vi "test Import Configuration File.vi"(8 "error in":errorcluster, 11 "TestCase in":refnum<class "Import.lvclass">) -> (0 "error out":errorcluster, 3 "TestCase out":refnum<class "Import.lvclass">)   [LabVIEW 2020, in "Import.lvclass"]
uses:
  Import.lvclass
  Import.lvclass/Import.ctl
  C:/Program Files/National Instruments/LabVIEW 2026/vi.lib/addons/_JKI Toolkits/VI Tester/TestCase.llb/TestCase.lvclass
  <vilib>/addons/_JKI Toolkits/VI Tester/TestCase.llb/TestCase.lvclass
  Import/ARINC 429 Import.lvlib
  <userlib>/_OpenG.lib/appcontrol/appcontrol.llb/openg_application_control.lvlib
  <vilib>/NI/VeriStand Custom Device Testing Tools/VeriStandTestUtilities/VeriStandTestUtilities.lvlib
  Shared/Transfer Type.ctl
  Shared/Direction.ctl
  Shared/Transfer Speed.ctl
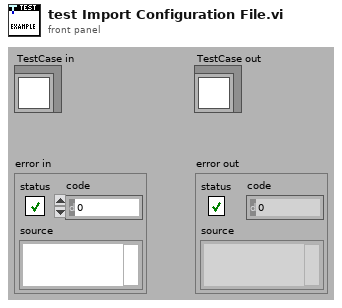
[diagram p1: front panel]
types:
  T1 = typedef "Direction.ctl" = enum16{"Rx", "Tx"}
  T2 = typedef "Transfer Type.ctl" = enum16{"Scheduled", "Acyclic", "Block", "Strobe"}
  T3 = typedef "Transfer Speed.ctl" = enum16{"LO (12.5 kb/s)", "HI (100 kb/s)"}
  T4 = cluster{"hardware channel":i32, "direction":T1, "labels":cluster{"label (Dec)":i32, "parameters":cluster{"name":string, "unit":string, "Parameter":cluster{"start index":i32, "size":i32, "encoding":enum16{"BNR", "BCD", "Discrete"}, "signed":bool, "scale multiplier":dbl, "scale offset":dbl, "default value":dbl}}[], "SDI value":u8, "SDI enabled":bool, "transfer type":T2, "SDI enabled 2":bool, "transmit period":u32}[], "speed":T3}[]
  T5 = typedef "VS Channels Definition for All Labels on Hardware Channel.ctl" = cluster{"hardware channel":i32, "direction":T1, "labels":T6[], "speed":T3}
  T6 = typedef "VS Channels Definition for Label.ctl" = cluster{"label (Dec)":u32, "parameters":T7[], "SDI value":u8, "SDI enabled":bool, "transfer type":T2, "create timestamp":bool, "transmit period":u32}
  T7 = typedef "VS Channel Definition for Parameter.ctl" = cluster{"name":string, "unit":string, "Parameter":T8}
  T8 = typedef "Parameter Definition.ctl" = cluster{"start index":i32, "size":i32, "encoding":T9, "signed":bool, "scale multiplier":dbl, "scale offset":dbl, "default value":dbl}
  T9 = typedef "Encoding and Decoding.lvlib/Encoding.ctl" = enum16{"BNR", "BCD", "Discrete"}
  T10 = cluster{"hardware channel":i32, "direction":T1, "labels":cluster{"label (Dec)":i32, "parameters":cluster{"name":string, "unit":string, "Parameter":cluster{"start index":i32, "size":i32, "encoding":enum16{"BNR", "BCD", "Discrete"}, "signed":bool, "scale multiplier":dbl, "scale offset":dbl, "default value":dbl}}[], "SDI value":u8, "SDI enabled":bool, "transfer type":T2, "SDI enabled 2":bool, "transmit period":u32}[], "speed":T3}
  T11 = cluster{"label (Dec)":i32, "parameters":cluster{"name":string, "unit":string, "Parameter":cluster{"start index":i32, "size":i32, "encoding":enum16{"BNR", "BCD", "Discrete"}, "signed":bool, "scale multiplier":dbl, "scale offset":dbl, "default value":dbl}}[], "SDI value":u8, "SDI enabled":bool, "transfer type":T2, "SDI enabled 2":bool, "transmit period":u32}[]
  T12 = cluster{"label (Dec)":i32, "parameters":cluster{"name":string, "unit":string, "Parameter":cluster{"start index":i32, "size":i32, "encoding":enum16{"BNR", "BCD", "Discrete"}, "signed":bool, "scale multiplier":dbl, "scale offset":dbl, "default value":dbl}}[], "SDI value":u8, "SDI enabled":bool, "transfer type":T2, "SDI enabled 2":bool, "transmit period":u32}
  T13 = cluster{"name":string, "unit":string, "Parameter":cluster{"start index":i32, "size":i32, "encoding":enum16{"BNR", "BCD", "Discrete"}, "signed":bool, "scale multiplier":dbl, "scale offset":dbl, "default value":dbl}}[]
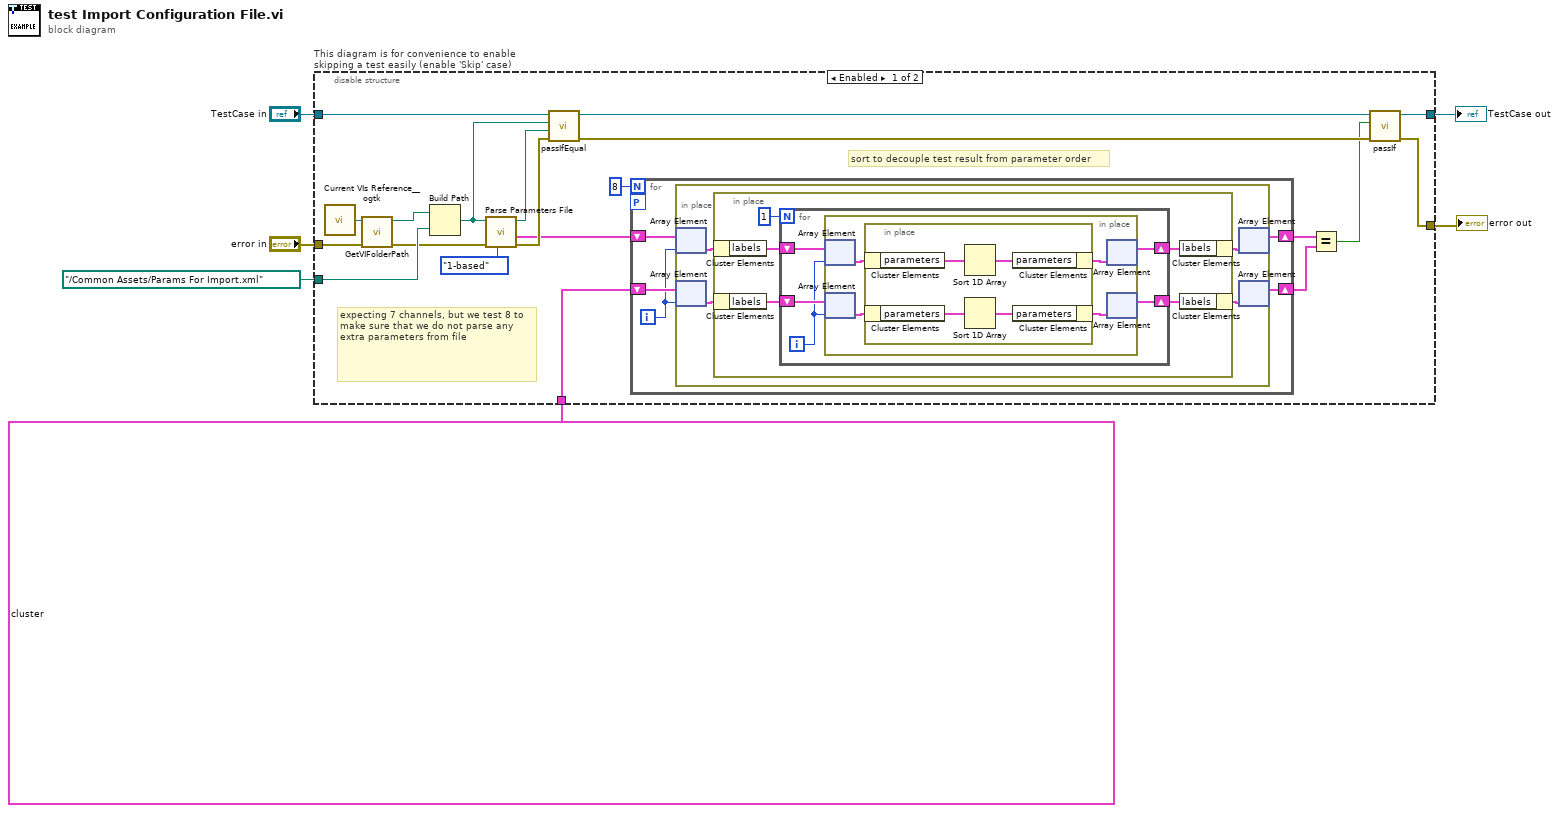
[diagram p0: block diagram]
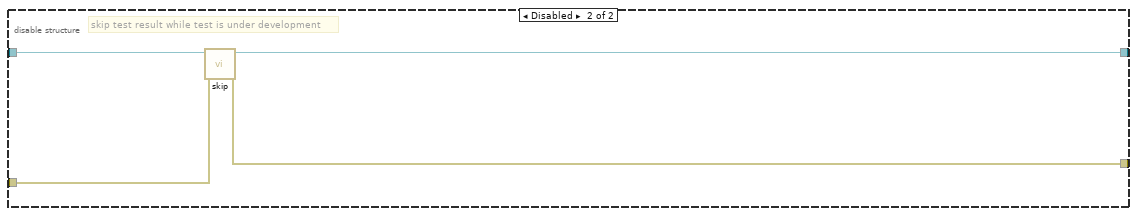
[diagram p2: hidden frame]
diagram:
  n1 = disable-structure "This diagram is for convenience to enable skipping a test easily (enable 'Skip' case)" shown="Enabled" {
    disable-tunnel: "TestCase in" -> [w26 w57]
    disable-tunnel: [w15 w55] -> w3
    disable-tunnel: [w16 w56] -> w5
    disable-tunnel: "error in" -> [w23 w54]
    disable-tunnel: path "../Common Assets/Params For Import.xml" ("Absolute or Relative Path") -> [w22 _]
    disable-tunnel: T4 [{"hardware channel"=1, "direction"=enum."Rx", "labels"=[{"label (Dec)"=134, "parameters"=[{"name"="Altitude_Rx", "unit"="psi", "Parameter"={"start index"=18, "size"=10, "encoding"=enum."BNR", "signed"=TRUE, "scale multiplier"=16.0, "scale offset"=0.0, "default value"=0.0}}, {"name"="SSM", "unit"="", "Parameter"={"start index"=29, "size"=2, "encoding"=enum."BNR", "signed"=FALSE, "scale multiplier"=1.0, "scale offset"=0.0, "default value"=0.0}}, {"name"="Parity", "unit"="", "Parameter"={"start index"=31, "size"=1, "encoding"=enum."Discrete", "signed"=FALSE, "scale multiplier"=1.0, "scale offset"=0.0, "default value"=0.0}}], "SDI value"=4, "SDI enabled"=FALSE, "transfer type"=enum."Scheduled", "SDI enabled 2"=TRUE, "transmit period"=1000}], "speed"=enum."LO (12.5 kb/s)"}, {"hardware channel"=2, "direction"=enum."Rx", "labels"=[{"label (Dec)"=135, "parameters"=[{"name"="Altitude_Rx", "unit"="ft", "Parameter"={"start index"=10, "size"=19, "encoding"=enum."BCD", "signed"=TRUE, "scale multiplier"=1.0, "scale offset"=0.0, "default value"=0.0}}, {"name"="SSM", "unit"="", "Parameter"={"start index"=29, "size"=2, "encoding"=enum."BNR", "signed"=FALSE, "scale multiplier"=1.0, "scale offset"=0.0, "default value"=0.0}}], "SDI value"=2, "SDI enabled"=TRUE, "transfer type"=enum."Scheduled", "SDI enabled 2"=FALSE, "transmit period"=1000}], "speed"=enum."HI (100 kb/s)"}, {"hardware channel"=4, "direction"=enum."Rx", "labels"=[{"label (Dec)"=136, "parameters"=[{"name"="Altitude_Rx", "unit"="m", "Parameter"={"start index"=13, "size"=16, "encoding"=enum."BNR", "signed"=TRUE, "scale multiplier"=1.0, "scale offset"=0.0, "default value"=0.0}}, {"name"="valid_Rx", "unit"="", "Parameter"={"start index"=10, "size"=1, "encoding"=enum."Discrete", "signed"=FALSE, "scale multiplier"=1.0, "scale offset"=0.0, "default value"=0.0}}, {"name"="current_Rx", "unit"="", "Parameter"={"start index"=11, "size"=1, "encoding"=enum."Discrete", "signed"=FALSE, "scale multiplier"=1.0, "scale offset"=0.0, "default value"=0.0}}, {"name"="SSM", "unit"="", "Parameter"={"start index"=29, "size"=2, "encoding"=enum."BNR", "signed"=FALSE, "scale multiplier"=1.0, "scale offset"=0.0, "default value"=0.0}}], "SDI value"=4, "SDI enabled"=FALSE, "transfer type"=enum."Scheduled", "SDI enabled 2"=FALSE, "transmit period"=1000}], "speed"=enum."HI (100 kb/s)"}, {"hardware channel"=17, "direction"=enum."Tx", "labels"=[{"label (Dec)"=134, "parameters"=[{"name"="Altitude_Tx", "unit"="psi", "Parameter"={"start index"=18, "size"=10, "encoding"=enum."BNR", "signed"=TRUE, "scale multiplier"=16.0, "scale offset"=0.0, "default value"=0.0}}], "SDI value"=4, "SDI enabled"=FALSE, "transfer type"=enum."Scheduled", "SDI enabled 2"=FALSE, "transmit period"=20000}], "speed"=enum."HI (100 kb/s)"}, {"hardware channel"=19, "direction"=enum."Tx", "labels"=[{"label (Dec)"=135, "parameters"=[{"name"="Altitude_Tx", "unit"="ft", "Parameter"={"start index"=10, "size"=19, "encoding"=enum."BCD", "signed"=TRUE, "scale multiplier"=1.0, "scale offset"=0.0, "default value"=0.0}}], "SDI value"=2, "SDI enabled"=TRUE, "transfer type"=enum."Scheduled", "SDI enabled 2"=FALSE, "transmit period"=50000}], "speed"=enum."HI (100 kb/s)"}, {"hardware channel"=21, "direction"=enum."Tx", "labels"=[{"label (Dec)"=136, "parameters"=[{"name"="Altitude_Tx", "unit"="m", "Parameter"={"start index"=13, "size"=16, "encoding"=enum."BNR", "signed"=TRUE, "scale multiplier"=1.0, "scale offset"=0.0, "default value"=0.0}}, {"name"="valid_Tx", "unit"="", "Parameter"={"start index"=10, "size"=1, "encoding"=enum."Discrete", "signed"=FALSE, "scale multiplier"=1.0, "scale offset"=0.0, "default value"=0.0}}, {"name"="current_Tx", "unit"="", "Parameter"={"start index"=11, "size"=1, "encoding"=enum."Discrete", "signed"=FALSE, "scale multiplier"=1.0, "scale offset"=0.0, "default value"=0.0}}], "SDI value"=4, "SDI enabled"=FALSE, "transfer type"=enum."Acyclic", "SDI enabled 2"=FALSE, "transmit period"=1000}], "speed"=enum."LO (12.5 kb/s)"}] ("ports") -> [w11 _]
    frame Enabled {
      # "sort to decouple test result from parameter order"
      # "expecting 7 channels, but we test 8 to make sure that we do not parse any extra parameters from file"
      n2 = call <userlib>:"Current VIs Reference__ogtk.vi"() -> ("Current VI's reference"=w25:refnum<vi>)  [unwired: 5 in]
      n3 = call <vilib>:"GetVIFolderPath.vi"("error in (no error)"=w23, "VI Reference in"=w25) -> ("error out"=w20:errorcluster, "VI Folder Path out"=w24:path)  [unwired: 8 in]
      n4 = Build Path(base path=w24, name or relative path=w22) -> (appended path=w21:path)
      n5 = call "Parse Parameters File.vi"("ch indexing (0-based)"=enum16{"0-based", "1-based"}."1-based", "error in"=w20, "path to XML document"=w21) -> ("error out"=w17:errorcluster, "ports"=w12:T5[], "path to XML document out"=w13:path)  [unwired: 6 in]
      n6 = call-dynamic "passIfEqual.vi"("error in (no error)"=w17, "y"=w13, "x"=w21, "TestCase in"=w26) -> ("error out"=w19:errorcluster, "TestCase out"=w18:refnum<class "Import.lvclass">)  [unwired: 6 in]
      n7 = for {
        N: 8 -> [_]
        shift-right: [w28] -> w10
        shift-left: w12 -> [w31]
        shift-right: [w27] -> w9
        shift-left: w11 -> [w30]
        workers-P: _ -> [_]
        i -> [w29]
        n8 = in-place {
          n9 = in-place-array #1(w31, w29) -> (w35:T5)
          n10 = in-place-array #2(w30, w29) -> (w34:T10)
          n11 = in-place {
            n12 = in-place-cluster #3(w35) -> ("labels"=w40:T6[])
            n13 = in-place-cluster #4(w34) -> ("labels"=w39:T11)
            n14 = for {
              N: 1 -> [_]
              shift-right: [w41] -> w38
              shift-left: w40 -> [w45]
              shift-right: [w42] -> w37
              shift-left: w39 -> [w44]
              i -> [w43]
              n15 = in-place {
                n16 = in-place-array #5(w45, w43) -> (w49:T6)
                n17 = in-place-array #6(w44, w43) -> (w48:T12)
                n18 = in-place {
                  n19 = in-place-cluster #7(w49) -> ("parameters"=w53:T7[])
                  n20 = in-place-cluster #8(w48) -> ("parameters"=w52:T13)
                  n21 = Sort 1D Array(array=w53) -> (sorted array=w51:T7[])
                  n22 = Sort 1D Array(array=w52) -> (sorted array=w50:T13)
                  n23 = in-place-cluster #7("parameters"=w51) -> (w47:T6)
                  n24 = in-place-cluster #8("parameters"=w50) -> (w46:T12)
                }
                n25 = in-place-array #5(w47) -> (w41:T6[])  [unwired: 1 out]
                n26 = in-place-array #6(w46) -> (w42:T11)  [unwired: 1 out]
              }
            }
            n27 = in-place-cluster #3("labels"=w38) -> (w33:T5)
            n28 = in-place-cluster #4("labels"=w37) -> (w32:T10)
          }
          n29 = in-place-array #1(w33) -> (w28:T5[])  [unwired: 1 out]
          n30 = in-place-array #2(w32) -> (w27:T4)  [unwired: 1 out]
        }
      }
      n31 = Equal?(x=w10, y=w9) -> (x = y?=w14:bool)
      n32 = call-dynamic "passIf.vi"("error in (no error)"=w19, "pass"=w14, "TestCase in"=w18) -> ("error out"=w16:errorcluster, "TestCase out"=w15:refnum<class "Import.lvclass">)  [unwired: 7 in]
    }
    frame Disabled {
      # "skip test result while test is under development"
      n33 = call <vilib>:"skip.vi"("error in (no error)"=w54, "TestCase in"=w57) -> ("error out"=w56:errorcluster, "TestCase out"=w55:refnum<class "Import.lvclass">)  [unwired: 8 in]
    }
  }
  "error out" <- w5
  "TestCase out" <- w3
